vi "HamamatsuFluor Buffer.vi"(6 "Image Type":T1=7 items=["Grayscale (U8)", "Grayscale (I16)", "Grayscale (SGL)", "Complex (CSG)", "RGB (U32)", "HSL (U32)", "RGB (U64)", "Grayscale (U16)"], 7 "Action":enum16{"Get", "Acquire", "Release"}(ring), 8 "error in (no error)":errorcluster, 9 "Image Height":u32, 10 "Image Width":u32, 11 "Buffer Length":u32) -> (0 "error out":errorcluster, 1 "Buffer Write Event":refnum<user-event>, 3 "Image Buffer Pointers":u64[](array[numeric]))   [LabVIEW 2020, in "DAQ Timed SPIM.lvlib" / "HamamatsuFluor_v2.lvlib"]
uses:
  HamamatsuFluor_v2.lvlib
  WIN Memory Map.llb/WIN MMAP.lvlib
panel:
  # "Each camera actor needs its own\ncopy of this VI"
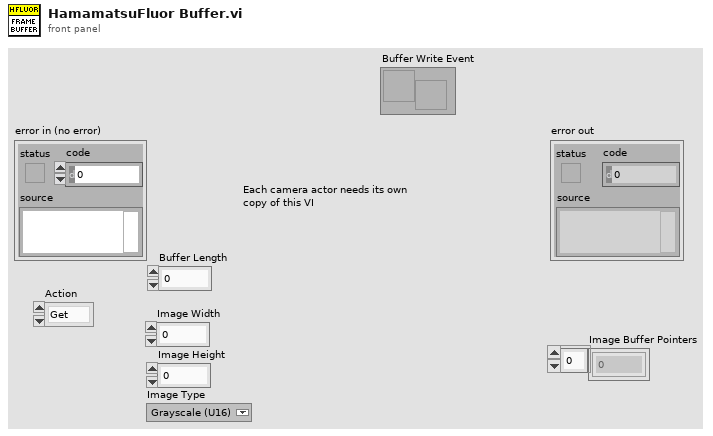
[diagram p1: front panel]
types:
  T1 = typedef "Image Type" = u32
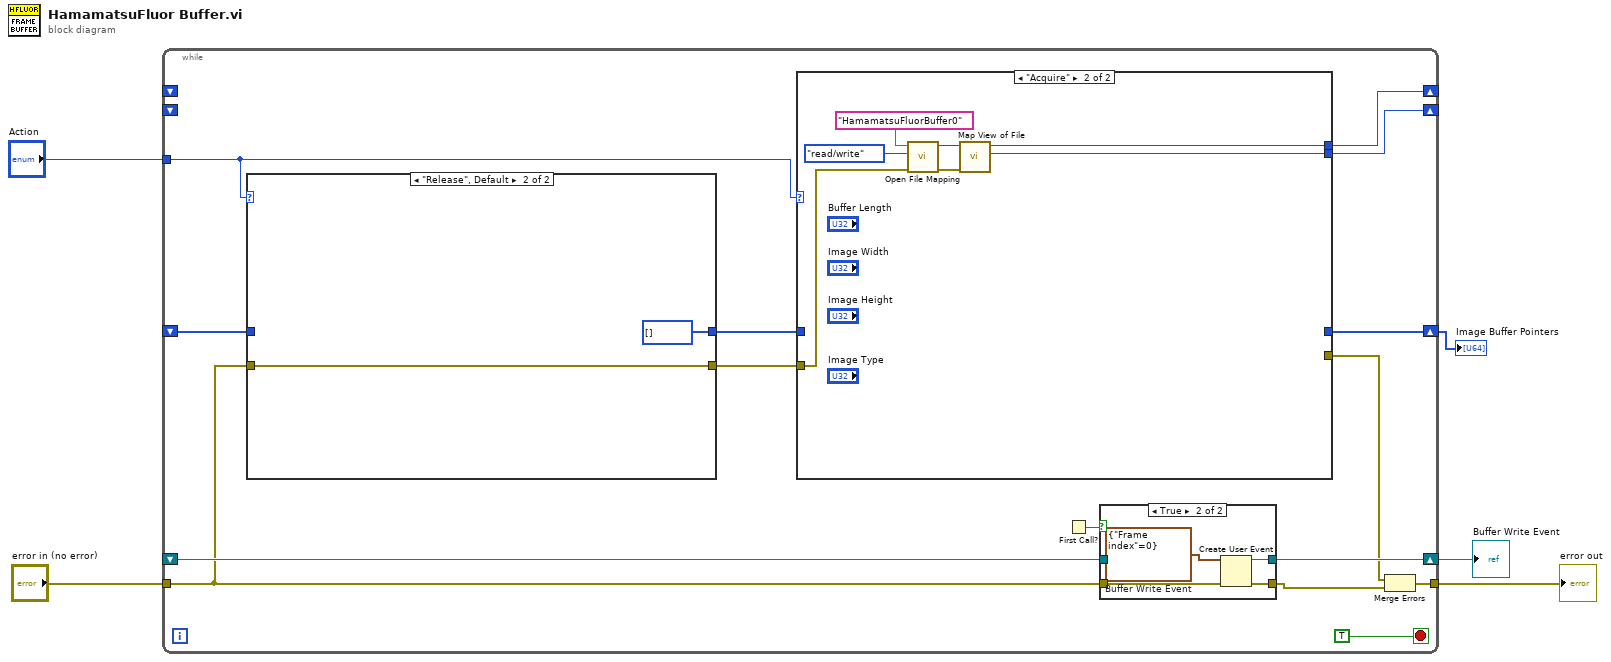
[diagram p0: block diagram]
diagram:
  n1 = while {
    tunnel: "error in (no error)" -> [w9]
    tunnel: [w15] -> w5
    shift-right: [w16] -> w2
    shift-left: _ -> [w10]
    shift-right: [w17] -> w1
    shift-left: _ -> [w18]
    tunnel: "Action" -> [w8]
    shift-right: [w7] -> _
    shift-left: _ -> [_]
    shift-right: [w6] -> _
    shift-left: _ -> [_]
    stop <- TRUE stop-if-true
    n2 = case shown="\"Release\", Default" w8 {
      tunnel: [w22 u64[] []] -> w11
      tunnel: w10 -> [w22 _]
      tunnel: [w21 w23] -> w12
      tunnel: w9 -> [w21 w23]
      frame "Get" {
      }
      frame "Release", Default {
      }
    }
    n3 = case shown="\"Acquire\"" w8 {
      tunnel: [w26 w39] -> w16
      tunnel: w11 -> [w26 _]
      tunnel: [w25 w38] -> w13
      tunnel: w12 -> [w25 w27]
      tunnel: [_ w30] -> w7
      tunnel: [_ w29] -> w6
      frame "Get", Default {
      }
      frame "Acquire" {
        n4 = call "Open File Mapping.vi"("error in (no error)"=w27, "access (0:read/write)"=enum16{"read/write", "read-only", "write-only"}."read/write", "map file name"="HamamatsuFluorBuffer0") -> ("error out"=w28:errorcluster, "handle"=w31:u64)  [unwired: 7 in]
        n5 = call "Map View of File.vi"("error in (no error)"=w28, "handle"=w31) -> ("startAddress"=w29:u64, "handle out"=w30:u64)  [unwired: 7 in, 1 out]
      }
    }
    n6 = First Call?() -> (First Call?: T/F=w19:bool)
    n7 = case shown="True" w19 {
      tunnel: [w40 w45] -> w17
      tunnel: [w41 w44] -> w14
      tunnel: w9 -> [w41 w43]
      tunnel: w18 -> [w40 _]
      frame False {
      }
      frame True {
        w42 = cluster{"Frame index":i32} {"Frame index"=0}  # Buffer Write Event
        n8 = Create User Event(user event datatype=w42, error in=w43) -> (user event=w45:refnum<user-event>, error out=w44:errorcluster)
      }
    }
    n9 = Merge Errors(w13, w14) -> (w15:errorcluster)
  }
  "error out" <- w5
  "Image Buffer Pointers" <- w2
  "Buffer Write Event" <- w1
